vi "Read Debug info.vi"(11 "CDebugInfo in":refnum<class "CDebugInfo.lvclass">) -> (1 "Debug info":string, 3 "CDebugInfo out":refnum<class "CDebugInfo.lvclass">)   [LabVIEW 2020, in "DependencyInspection.lvlib" / "CDebugInfo.lvclass"]
uses:
  CDebugInfo.lvclass
  CDebugInfo.lvclass/CDebugInfo.ctl
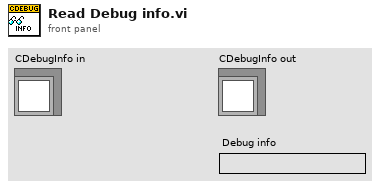
[diagram p1: front panel]
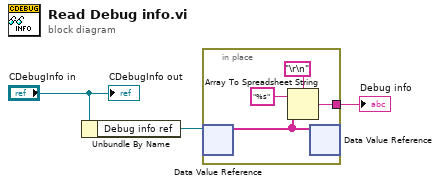
[diagram p0: block diagram]
diagram:
  n1 = Unbundle By Name("CDebugInfo in") -> ("Debug info ref"=w2:refnum<data-value>)
  n2 = in-place {
    in-place-border: [w4] -> w1
    n3 = in-place-dvr #1(w2) -> (w5:string[])  [unwired: 1 out]
    n4 = Array To Spreadsheet String(delimiter (Tab)="\r\n", array=w5, 3:"%s" ("format string")) -> (spreadsheet string=w4:string)
    n5 = in-place-dvr #1(w5) -> ()  [unwired: 2 out]
  }
  "Debug info" <- w1
  "CDebugInfo out" <- "CDebugInfo in"
